vi "KY Device Info.vi"(8 "error in (no error)":errorcluster, 11 "index":i32) -> (0 "error out":errorcluster)   [LabVIEW 2023]
doc: "KYFG_API FGSTATUS KYFG_CameraScan(FGHANDLE handle, CAMHANDLE *camHandleArray, int *detectedCameras);"
uses:
  KYFGLib_lv.lvlib
  KYFGLib.dll
panel:
  out "KY_DEVICE_INFO_OUT":T1
  out "error out 2":errorcluster
  in  "error in (no error) 2":errorcluster
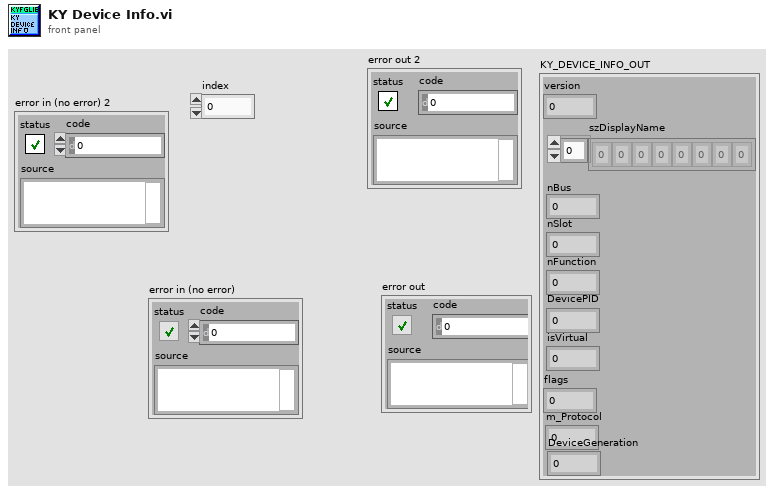
[diagram p1: front panel]
types:
  T1 = cluster{"version":u32, "szDisplayName":u8[], "isVirtual":u8, "DevicePID":u32, "nFunction":i32, "nSlot":i32, "nBus":u32, "flags":u8, "m_Protocol":u32, "DeviceGeneration":u32}
  T2 = cluster{"version":u32, "szDisplayName":u8[], "nBus":i32, "nSlot":i32, "nFunction":i32, "DevicePID":u32, "isVirtual":u8, "flags":u8, "m_Protocol":u32, "DeviceGeneration":u32}
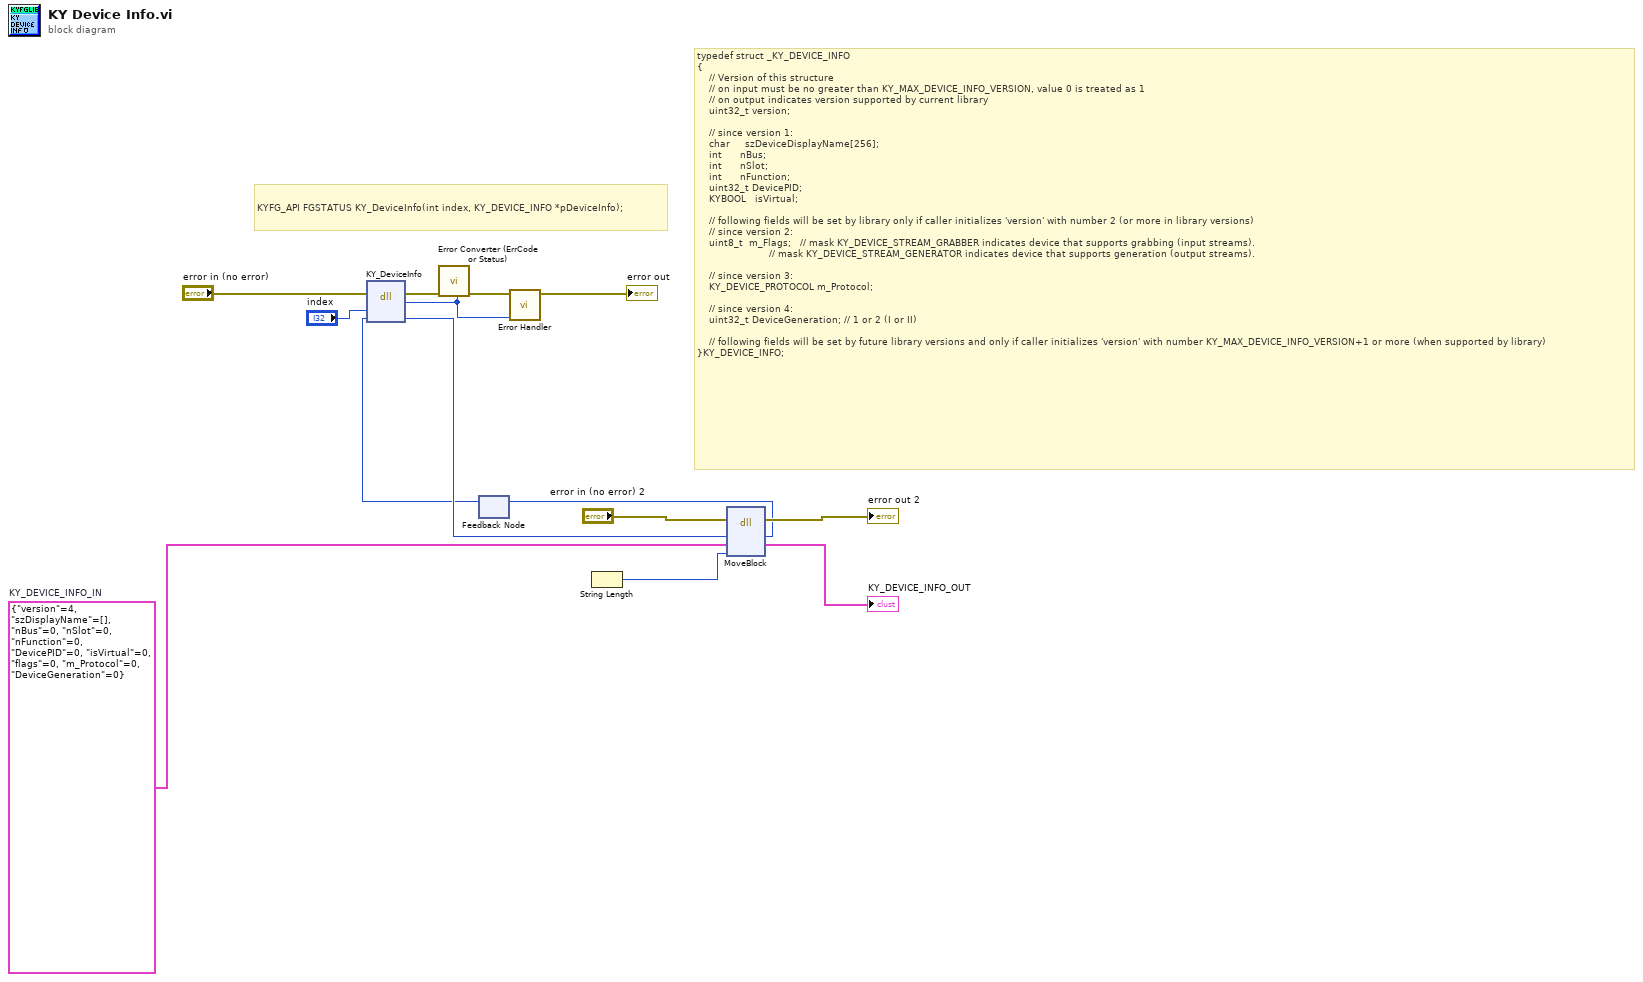
[diagram p0: block diagram]
diagram:
  w4 = T2 {"version"=4, "szDisplayName"=[], "nBus"=0, "nSlot"=0, "nFunction"=0, "DevicePID"=0, "isVirtual"=0, "flags"=0, "m_Protocol"=0, "DeviceGeneration"=0}  # KY_DEVICE_INFO_IN
  # "typedef struct _KY_DEVICE_INFO\n{\n    // Version of this structure\n    // on input must be no greater than KY_MAX_DEVICE_INFO_VERSION, value 0 is treated as 1\n    // on output indicates version supported by current library\n    uint32_t version;\n\n    // since version 1:\n    char     szDeviceDisplayName[256];\n    int      nBus;\n    int      nSlot;\n    int      nFunction;\n    uint32_t DevicePID;\n    KYBOOL   isVirtual;\n\n    // following fields will be set by library only if caller initializes 'version' with number 2 (or more in library versions)\n    // since version 2:\n    uint8_t  m_Flags;   // mask KY_DEVICE_STREAM_GRABBER indicates device that supports grabbing (input streams).\n                        // mask KY_DEVICE_STREAM_GENERATOR indicates device that supports generation (output streams).\n\n    // since version 3:\n    KY_DEVICE_PROTOCOL m_Protocol;\n\n    // since version 4:\n    uint32_t DeviceGeneration; // 1 or 2 (I or II)\n\n    // following fields will be set by future library versions and only if caller initializes 'version' with number KY_MAX_DEVICE_INFO_VERSION+1 or more (when supported by library)\n}KY_DEVICE_INFO;"
  # "KYFG_API FGSTATUS KY_DeviceInfo(int index, KY_DEVICE_INFO *pDeviceInfo);"
  n1 = feedback #1() -> (w1:i32)  [unwired: 1 in]
  n2 = dll-call lib="KYFGLib.dll" fn="KY_DeviceInfo"(error in="error in (no error)", "index"="index", w1) -> (error out=w12:errorcluster, "return type"=w9:u32, w3:i32)  [unwired: 3 in, 1 out]
  n3 = call "Error Converter (ErrCode or Status).vi"("error in (no error)"=w12, "error code"=w9) -> ("error out"=w11:errorcluster)  [unwired: 9 in]
  n4 = call "Error Handler.vi"("Return Code"=w9, "Error In"=w11) -> ("Error Out"=→"error out":errorcluster)  [unwired: 9 in]
  n5 = String Length() -> (length=w7:i32)  [unwired: 1 in]
  n6 = dll-call lib="LabVIEW" fn="MoveBlock"(error in="error in (no error) 2", "ps"=w3, "pd"=w4, "size"=w7) -> (error out=→"error out 2":errorcluster, "ps"=w2:i32, "pd"=→"KY_DEVICE_INFO_OUT":T2)  [unwired: 3 in, 2 out]
  n7 = feedback-in #1(w2) -> ()
